vi "GPIB_SR400_1.vi"() -> (2 "output array":string[][](array[string]))   [LabVIEW 2024]
uses:
  <vilib>/Utility/error.llb/Trim Whitespace One-Sided.vi
panel:
  out "output array 3":string[][](array[string])
  out "output array 2":string[](array[string])
  out "# of loop":i32
  out "Current Value":string[](array[string])
  out "Waveform Chart":i32(graph)
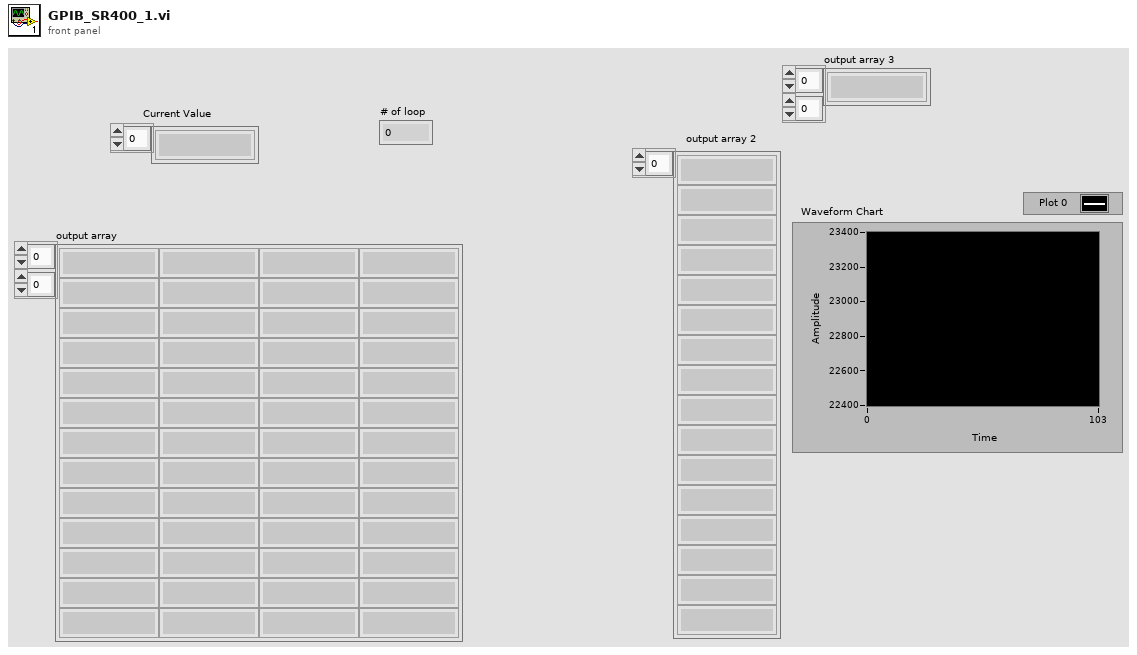
[diagram p1: front panel]
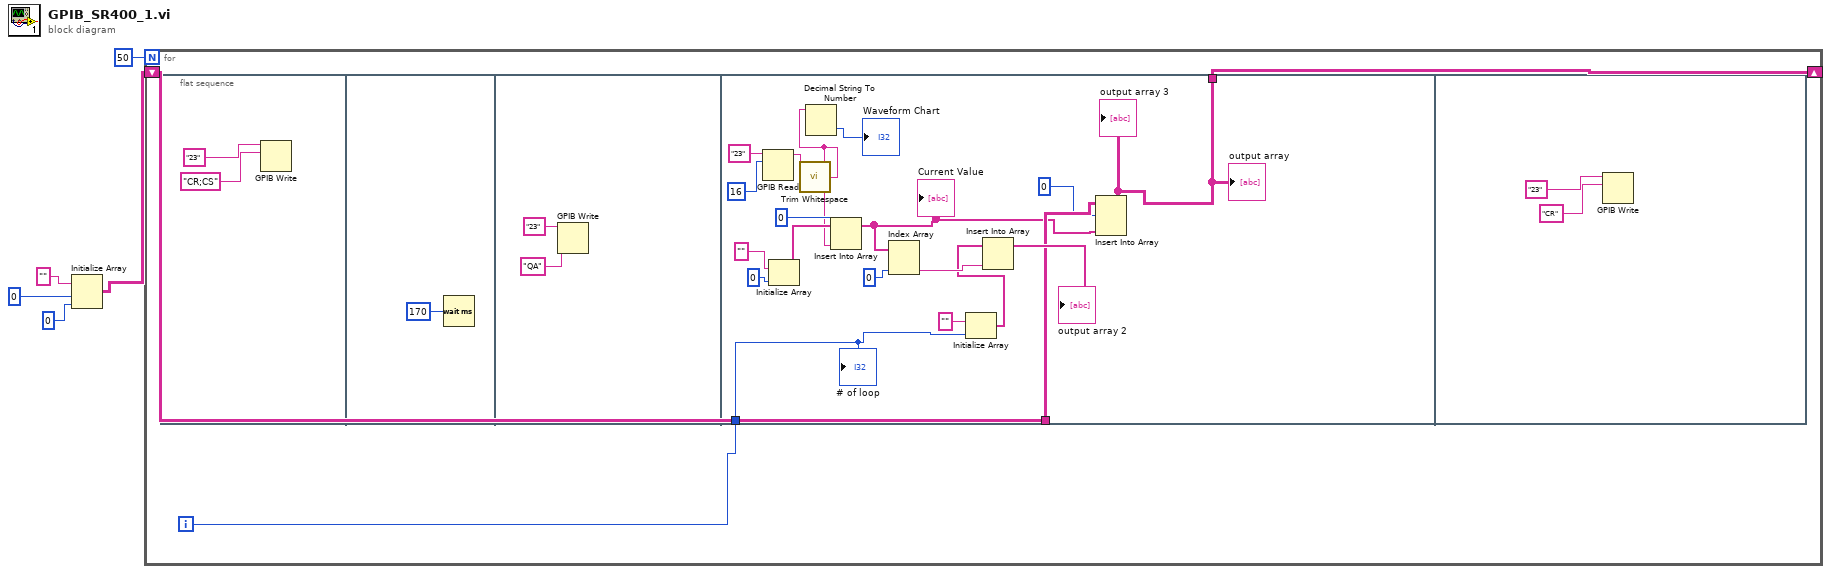
[diagram p0: block diagram]
diagram:
  n1 = Initialize Array("", 0 ("dimension size"), 0 ("dimension size")) -> (w1:string[][])
  n2 = for {
    N: 50 -> [_]
    shift-right: [w8] -> _
    shift-left: w1 -> [w6]
    i -> [w7]
    n3 = flat-sequence {
      tunnel: w7 -> [w19]
      tunnel: w6 -> [w20]
      tunnel: [w16] -> w8
      frame #0 {
        n4 = GPIB Write(0:"23" ("address string"), 1:"CR;CS" ("data")) -> ()  [unwired: 3 in, 2 out]
      }
      frame #1 {
        n5 = Wait (ms)(milliseconds to wait=u32 170) -> ()  [unwired: 1 out]
      }
      frame #2 {
        n6 = GPIB Write(0:"23" ("address string"), 1:"QA" ("data")) -> ()  [unwired: 3 in, 2 out]
      }
      frame #3 {
        n7 = GPIB Read(0:"23" ("address string"), 1:16 ("byte count")) -> (5:w15:string)  [unwired: 3 in, 2 out]
        n8 = Initialize Array("", 0 ("dimension size")) -> (w28:string[])
        n9 = call <vilib>:"Trim Whitespace.vi"("string"=w15) -> ("trimmed string"=w14:string)  [unwired: 1 in]
        n10 = Decimal String To Number(string=w14) -> (number=→"Waveform Chart":i32)  [unwired: 2 in, 1 out]
        n11 = Insert Into Array "Insert Into Array"(array=w28, index=0, new element=w14) -> (w17:string[])
        "Current Value" <- w17
        n12 = Index Array "Index Array"(array=w17, index #2=0 ("index")) -> (element #2=w24:string)  [unwired: 1 in, 1 out]
        n13 = Initialize Array("", w19) -> (w22:string[])
        n14 = Insert Into Array "Insert Into Array"(array=w22, new element=w24) -> (→"output array 2":string[])  [unwired: 1 in]
        n15 = Insert Into Array "Insert Into Array"(array=w20, index (row)=0 ("index"), new element=w17) -> (w16:string[][])  [unwired: 1 in]
        "output array 3" <- w16
        "output array" <- w16
        "# of loop" <- w19
      }
      frame #4 {
        n16 = GPIB Write(0:"23" ("address string"), 1:"CR" ("data")) -> ()  [unwired: 3 in, 2 out]
      }
    }
  }
